vi "Launch Root Actor_Actor_Generates Actor Traces.vi"() -> ()   [LabVIEW 2020]
uses:
  <vilib>/addons/_JKI Toolkits/Caraya/classes/Test/Test.lvclass
  <vilib>/addons/_JKI Toolkits/Caraya/classes/Assert/Assert.lvclass
  ActorFramework/Actor/Actor.lvclass
  Test Harness/AF Trace Queue/AF Trace Queue.lvclass
  ActorFramework/Stop Msg/Stop Msg.lvclass
  <vilib>/addons/_JKI Toolkits/Caraya/classes/Assert/Assert Equal Value_Variant.vi
panel:
  out "Array":string[](array[string])
  out "error out":errorcluster
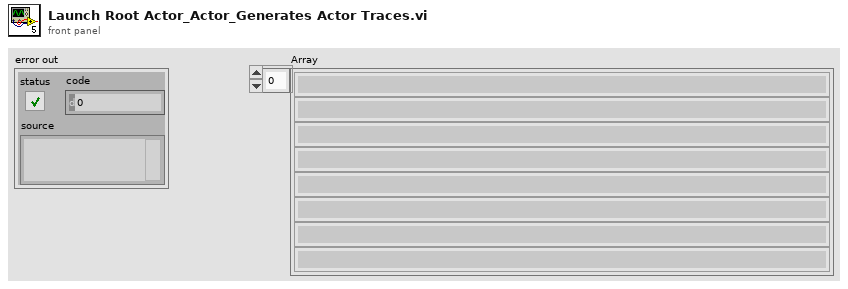
[diagram p1: front panel]
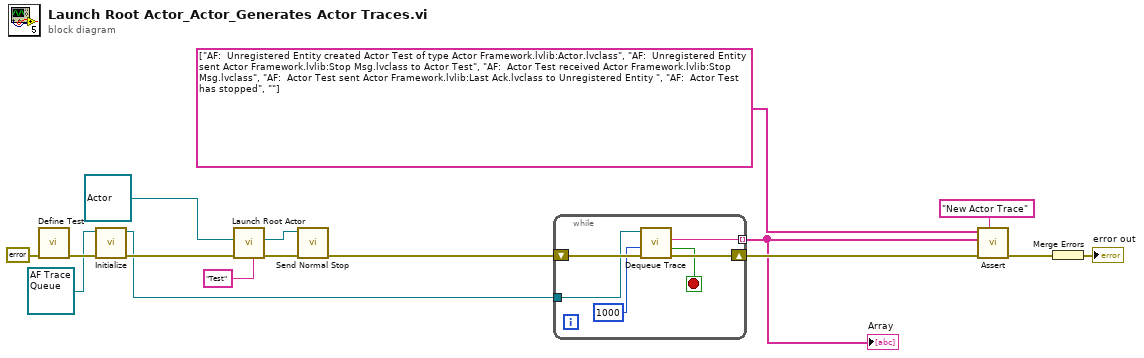
[diagram p0: block diagram]
diagram:
  n1 = call <vilib>:"Define Test.vi"("error in (no error)"=errorcluster {"status"=FALSE, "code"=0, "source"=""}) -> ("error out"=w15:errorcluster)  [unwired: 9 in, 1 out]
  n2 = call-dynamic "Initialize.vi"("error in (no error)"=w15, "AF Trace Queue in"=refnum<class "AF Trace Queue.lvclass"> refnum) -> ("error out"=w13:errorcluster, "AF Trace Queue out"=w8:refnum<class "AF Trace Queue.lvclass">)  [unwired: 8 in]
  n3 = call "Launch Root Actor.vi"("Debug Alias"="Test", "error in (no error)"=w13, "Actor"=refnum<class "Actor.lvclass"> refnum ("Actor Framework:Actor")) -> ("error out"=w12:errorcluster, "Actor's Enqueuer"=w10:refnum<class "Message Enqueuer.lvclass">)  [unwired: 7 in]
  n4 = call "Send Normal Stop.vi"("error in (no error)"=w12, "Message Enqueuer"=w10) -> ("error out"=w11:errorcluster)  [unwired: 9 in]
  n5 = while {
    tunnel: w8 -> [w21]
    shift-right: [w20] -> w6
    shift-left: w11 -> [w22]
    tunnel: [w17] -> w4 mode=indexing
    stop <- w18 stop-if-true
    n6 = call "Dequeue Trace.vi"("error in (no error)"=w22, "timeout in ms (-1)"=1000, "AF Trace Queue in"=w21) -> ("error out"=w20:errorcluster, "timed out?"=w18:bool, "Trace String"=w17:string)  [unwired: 5 in, 1 out]
  }
  "Array" <- w4
  n7 = call-poly <vilib>:"Assert.vi"("Label"="New Actor Trace" ("Label (VI Title)"), "error in (no error)"=w6, "Y"=w4, "X"=string[] ["AF:  Unregistered Entity created Actor Test of type Actor Framework.lvlib:Actor.lvclass", "AF:  Unregistered Entity sent Actor Framework.lvlib:Stop Msg.lvclass to Actor Test", "AF:  Actor Test received Actor Framework.lvlib:Stop Msg.lvclass", "AF:  Actor Test sent Actor Framework.lvlib:Last Ack.lvclass to Unregistered Entity ", "AF:  Actor Test has stopped", ""] ("Array")) -> ("error out"=w5:errorcluster)  [unwired: 6 in, 1 out]
  n8 = Merge Errors(w5) -> (→"error out":errorcluster)
